vi "Write Ex.vi"(8 "error in (no error)":errorcluster, 9 "DATOS":u8[](array[numeric]), 10 "PID":u32, 11 "VID":u32) -> (0 "error out":errorcluster, 3 "OUT":i32)   [LabVIEW 2011, in "HID_ARZ.lvlib"]
doc: "WRITE_EX WriteEx;"
uses:
  HID_ARZ.lvlib
  <userlib>/HID_ARZ/mcHID.dll
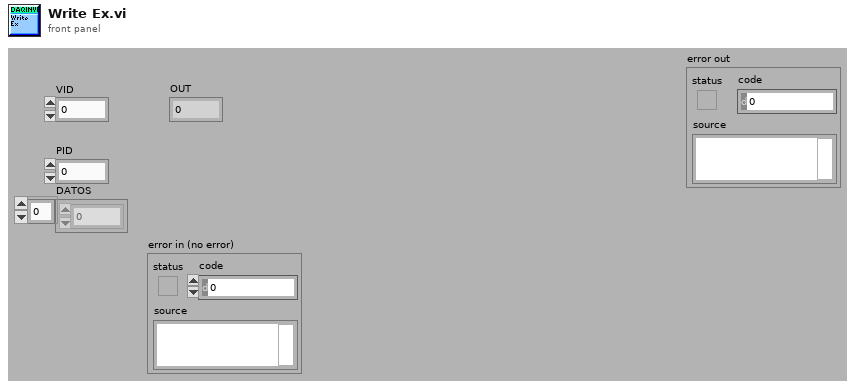
[diagram p1: front panel]
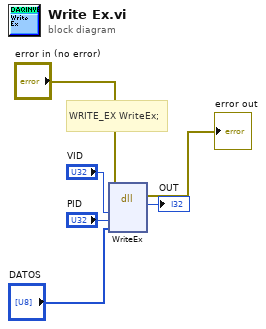
[diagram p0: block diagram]
diagram:
  # "WRITE_EX WriteEx;"
  n1 = dll-call lib="C:/Program Files (x86)/National Instruments/LabVIEW 2017/user.lib/HID_ARZ/mcHID.*" fn="WriteEx"(error in="error in (no error)", "VID"="VID", "PID"="PID", "DATOS"="DATOS") -> (error out=→"error out":errorcluster, "return type"=→"OUT":i32)  [unwired: 5 in, 1 out]
